vi "AddToGroupHelper.vi"(8 "error in (no error)":errorcluster, 9 "Group":string, 10 "Name":string, 11 "Setting Database in":refnum<class "Setting Database.lvclass">) -> (0 "error out":errorcluster, 2 "Active?":bool, 3 "Setting Database out":refnum<class "Setting Database.lvclass">)   [LabVIEW 2019, in "Setting Database.lvclass"]
uses:
  Setting Database.lvclass
  Path Settings/Path Settings.lvclass
  Rectangle Settings/Rectangle Settings.lvclass
  Funnel Settings/Funnel Settings.lvclass
  Dot Settings/Dot Settings.lvclass
  Identity/Identifier.lvclass
  C:/Users/Albro/Documents/GitHub/AFM-Lithography/lvsrc/Classes/Settings/ObjectSettings/ObjectSettings.lvclass
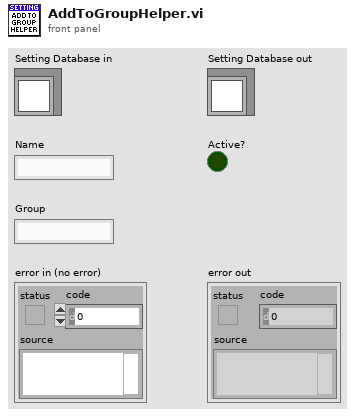
[diagram p1: front panel]
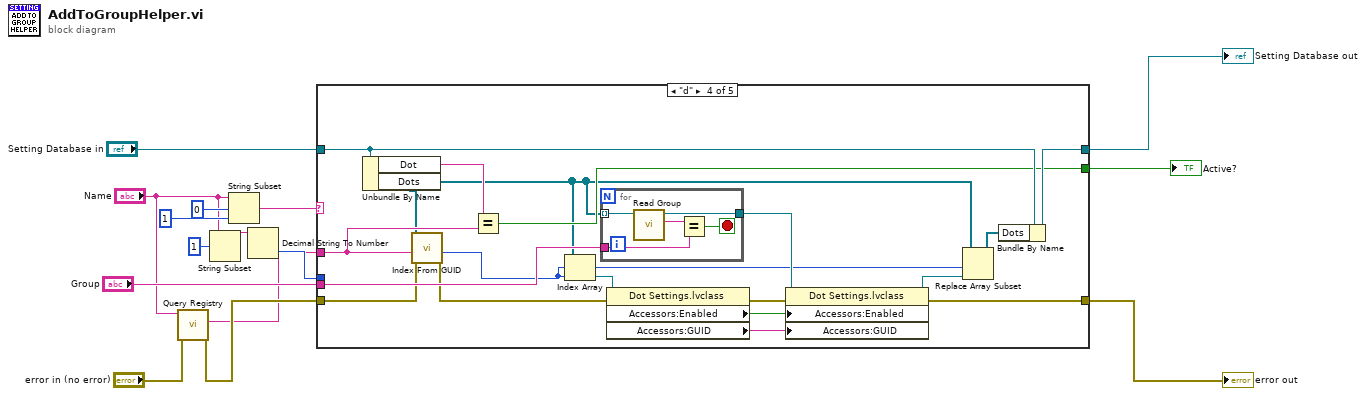
[diagram p0: block diagram]
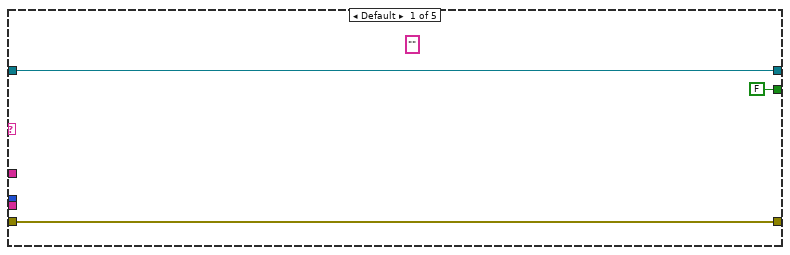
[diagram p2: hidden frame]
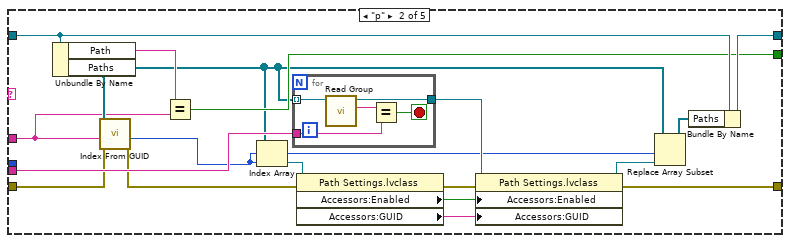
[diagram p3: hidden frame]
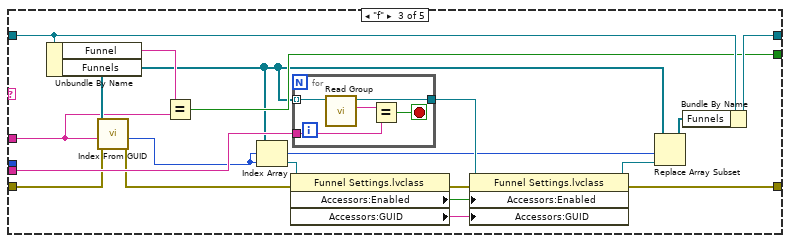
[diagram p4: hidden frame]
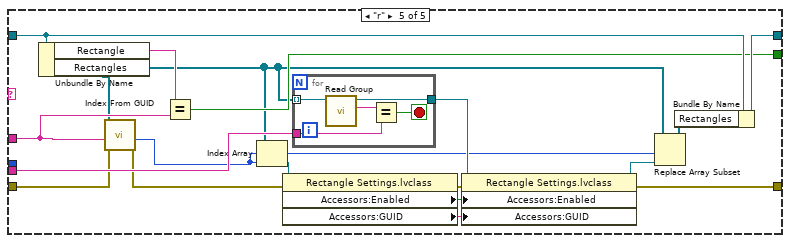
[diagram p5: hidden frame]
diagram:
  n1 = call "Query Registry.vi"("error in"="error in (no error)", "Name In"="Name") -> ("error out"=w3:errorcluster, "Alias"=w1:string)  [unwired: 6 in, 2 out]
  n2 = String Subset(string="Name", offset (0)=1) -> (substring=w13:string)  [unwired: 1 in]
  n3 = String Subset(string="Name", offset (0)=0, length (rest)=1 ("length (rest)")) -> (substring=w12:string)
  n4 = Decimal String To Number(string=w13) -> (number=w11:i32)  [unwired: 2 in, 1 out]
  n5 = case shown="\"d\"" w12 {
    tunnel: "Setting Database in" -> [w18 w35 w58 w81 w104]
    tunnel: [w18 w36 w59 w82 w105] -> w9
    tunnel: w11 -> [_ _ _ _ _]
    tunnel: [w17 w29 w52 w75 w98] -> w8
    tunnel: w3 -> [w17 w19 w44 w66 w88]
    tunnel: "Group" -> [_ w33 w56 w79 w102]
    tunnel: [FALSE w25 w48 w71 w94] -> w5
    tunnel: w1 -> [_ w22 w42 w69 w92]
    frame Default {
      (unwired) "" ("States Out")
    }
    frame "p" {
      n6 = Unbundle By Name(w35) -> ("Path"=w24:string, "Paths"=w23:refnum<class "Path Settings.lvclass">[])
      n7 = call "Index From GUID.vi"("error in"=w19, "GUID"=w22, "Objects In"=w23) -> ("error out"=w20:errorcluster, "Index"=w21:i32)  [unwired: 5 in, 2 out]
      n8 = Equal?(x=w24, y=w22) -> (x = y?=w25:bool)
      n9 = Index Array(array=w23, index=w21) -> (element=w31:refnum<class "Path Settings.lvclass">)
      n10 = for {
        tunnel: w23 -> [w41] mode=indexing
        tunnel: w33 -> [w39]
        tunnel: [w37] -> w26
        stop <- w38 stop-if-true
        n11 = call-dynamic "Read Group.vi"("ObjectSettings in"=w41) -> ("Group"=w40:string, "ObjectSettings out"=w37:refnum<class "Path Settings.lvclass">)  [unwired: 8 in, 1 out]
        n12 = Equal?(x=w40, y=w39) -> (x = y?=w38:bool)
      }
      n13 = property class="Path Settings.lvclass"(reference=w31, error in=w20) -> (error out=w30:errorcluster, "Accessors:Enabled"=w28:bool, "Accessors:GUID"=w32:string)  [unwired: 1 out]
      n14 = property class="Path Settings.lvclass"(reference=w26, error in=w30, "Accessors:Enabled"=w28, "Accessors:GUID"=w32) -> (reference out=w27:refnum<class "Path Settings.lvclass">, error out=w29:errorcluster)
      n15 = Replace Array Subset(array=w23, new element=w27, index=w21) -> (w34:refnum<class "Path Settings.lvclass">[])
      n16 = Bundle By Name(cluster=w35, "Paths"=w34) -> (w36:refnum<class "Setting Database.lvclass">)
    }
    frame "f" {
      n17 = Unbundle By Name(w58) -> ("Funnel"=w47:string, "Funnels"=w46:refnum<class "Funnel Settings.lvclass">[])
      n18 = call "Index From GUID.vi"("error in"=w44, "GUID"=w42, "Objects In"=w46) -> ("error out"=w45:errorcluster, "Index"=w43:i32)  [unwired: 5 in, 2 out]
      n19 = Equal?(x=w47, y=w42) -> (x = y?=w48:bool)
      n20 = Index Array(array=w46, index=w43) -> (element=w54:refnum<class "Funnel Settings.lvclass">)
      n21 = property class="Funnel Settings.lvclass"(reference=w54, error in=w45) -> (error out=w53:errorcluster, "Accessors:Enabled"=w51:bool, "Accessors:GUID"=w55:string)  [unwired: 1 out]
      n22 = for {
        tunnel: w46 -> [w64] mode=indexing
        tunnel: w56 -> [w62]
        tunnel: [w60] -> w49
        stop <- w61 stop-if-true
        n23 = call-dynamic "Read Group.vi"("ObjectSettings in"=w64) -> ("Group"=w63:string, "ObjectSettings out"=w60:refnum<class "Funnel Settings.lvclass">)  [unwired: 8 in, 1 out]
        n24 = Equal?(x=w63, y=w62) -> (x = y?=w61:bool)
      }
      n25 = property class="Funnel Settings.lvclass"(reference=w49, error in=w53, "Accessors:Enabled"=w51, "Accessors:GUID"=w55) -> (reference out=w50:refnum<class "Funnel Settings.lvclass">, error out=w52:errorcluster)
      n26 = Replace Array Subset(array=w46, new element=w50, index=w43) -> (w57:refnum<class "Funnel Settings.lvclass">[])
      n27 = Bundle By Name(cluster=w58, "Funnels"=w57) -> (w59:refnum<class "Setting Database.lvclass">)
    }
    frame "d" {
      n28 = Unbundle By Name(w81) -> ("Dot"=w70:string, "Dots"=w65:refnum<class "Dot Settings.lvclass">[])
      n29 = call "Index From GUID.vi"("error in"=w66, "GUID"=w69, "Objects In"=w65) -> ("error out"=w67:errorcluster, "Index"=w68:i32)  [unwired: 5 in, 2 out]
      n30 = Equal?(x=w70, y=w69) -> (x = y?=w71:bool)
      n31 = Index Array(array=w65, index=w68) -> (element=w77:refnum<class "Dot Settings.lvclass">)
      n32 = for {
        tunnel: w65 -> [w87] mode=indexing
        tunnel: w79 -> [w85]
        tunnel: [w83] -> w72
        stop <- w84 stop-if-true
        n33 = call-dynamic "Read Group.vi"("ObjectSettings in"=w87) -> ("Group"=w86:string, "ObjectSettings out"=w83:refnum<class "Dot Settings.lvclass">)  [unwired: 8 in, 1 out]
        n34 = Equal?(x=w86, y=w85) -> (x = y?=w84:bool)
      }
      n35 = property class="Dot Settings.lvclass"(reference=w77, error in=w67) -> (error out=w76:errorcluster, "Accessors:Enabled"=w74:bool, "Accessors:GUID"=w78:string)  [unwired: 1 out]
      n36 = property class="Dot Settings.lvclass"(reference=w72, error in=w76, "Accessors:Enabled"=w74, "Accessors:GUID"=w78) -> (reference out=w73:refnum<class "Dot Settings.lvclass">, error out=w75:errorcluster)
      n37 = Replace Array Subset(array=w65, new element=w73, index=w68) -> (w80:refnum<class "Dot Settings.lvclass">[])
      n38 = Bundle By Name(cluster=w81, "Dots"=w80) -> (w82:refnum<class "Setting Database.lvclass">)
    }
    frame "r" {
      n39 = Unbundle By Name(w104) -> ("Rectangle"=w93:string, "Rectangles"=w90:refnum<class "Rectangle Settings.lvclass">[])
      n40 = call "Index From GUID.vi"("error in"=w88, "GUID"=w92, "Objects In"=w90) -> ("error out"=w89:errorcluster, "Index"=w91:i32)  [unwired: 5 in, 2 out]
      n41 = Equal?(x=w93, y=w92) -> (x = y?=w94:bool)
      n42 = Index Array(array=w90, index=w91) -> (element=w100:refnum<class "Rectangle Settings.lvclass">)
      n43 = property class="Rectangle Settings.lvclass"(reference=w100, error in=w89) -> (error out=w99:errorcluster, "Accessors:Enabled"=w97:bool, "Accessors:GUID"=w101:string)  [unwired: 1 out]
      n44 = for {
        tunnel: w90 -> [w110] mode=indexing
        tunnel: w102 -> [w108]
        tunnel: [w106] -> w95
        stop <- w107 stop-if-true
        n45 = call-dynamic "Read Group.vi"("ObjectSettings in"=w110) -> ("Group"=w109:string, "ObjectSettings out"=w106:refnum<class "Rectangle Settings.lvclass">)  [unwired: 8 in, 1 out]
        n46 = Equal?(x=w109, y=w108) -> (x = y?=w107:bool)
      }
      n47 = property class="Rectangle Settings.lvclass"(reference=w95, error in=w99, "Accessors:Enabled"=w97, "Accessors:GUID"=w101) -> (reference out=w96:refnum<class "Rectangle Settings.lvclass">, error out=w98:errorcluster)
      n48 = Replace Array Subset(array=w90, new element=w96, index=w91) -> (w103:refnum<class "Rectangle Settings.lvclass">[])
      n49 = Bundle By Name(cluster=w104, "Rectangles"=w103) -> (w105:refnum<class "Setting Database.lvclass">)
    }
  }
  "error out" <- w8
  "Setting Database out" <- w9
  "Active?" <- w5
